vi "GpuMat Create.vi"(8 "error in (no error)":errorcluster) -> (0 "error out":errorcluster, 3 "GpuMat out":refnum<class "GpuMat.lvclass">)   [LabVIEW 2020, in "OpenLvVision_OpenCv.lvlib" / "Cuda.lvlib" / "GpuMat.lvclass"]
doc: "Object by reference!\n\nInitializes an empty `GpuMat`. This acts as a default constructor. It does not allocate any GPU memory; it simply creates the header structure. The matrix will have 0 rows and 0 columns, and its `.empty()` method will return true until data is uploaded or allocated to it."
uses:
  GpuMat.lvclass
  C:/Users/lukas/Documents/OpenLvVision_OpenCv/SourceCode/LabView/OpenLvVision_OpenCv/_LvHelpers/EdvrObject/EdvrObject.lvclass
  _LvHelpers/EdvrObject/TypeDef/Edvr.ctl
  _LvHelpers/EdvrObject/EdvrObject.lvclass/EdvrObject.ctl
  _LvHelpers/EdvrObject/EdvrObject.lvclass
  OpenLvVision_OpenCv.lvlib
  <vilib>/Utility/error.llb/Error Cluster From Error Code.vi
  <vilib>/ErrorRing/Error Ring.xnode
  Dlls/OlvOpenCvWrapper.dll
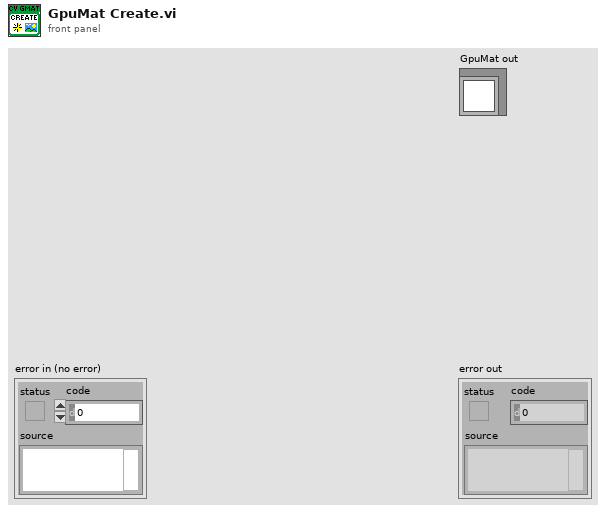
[diagram p1: front panel]
types:
  T1 = typedef "OpenLvVision_OpenCv.lvlib/EdvrObject.lvclass/Edvr.ctl" = refnum<data-value>
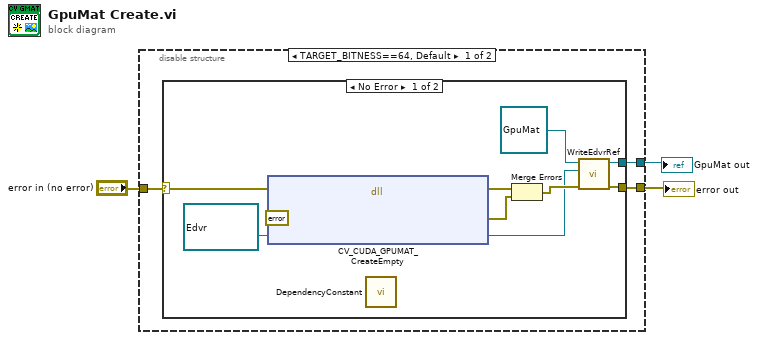
[diagram p0: block diagram]
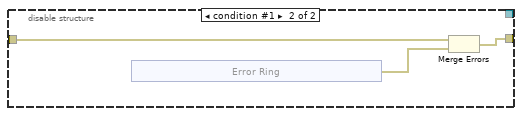
[diagram p3: hidden frame]
diagram:
  n1 = disable-structure shown="TARGET_BITNESS==64, Default" {
    disable-tunnel: "error in (no error)" -> [w6 w19]
    disable-tunnel: [w5 _] -> w2
    disable-tunnel: [w4 w20] -> w3
    frame condition #0 (active) {
      n2 = case shown="No Error" w6 {
        selector: w6 -> [w9 w17]
        tunnel: [w16 w17] -> w4
        tunnel: [w15 _] -> w5
        frame No Error {
          n3 = dll-call lib="C:/Users/lukas/Documents/OpenLvVision_OpenCv/SourceCode/LabView/OpenLvVision_OpenCv/Dlls/OlvOpenCvWrapper.dll" fn="CV_CUDA_GPUMAT_CreateEmpty"(error in=w9, "Error"=errorcluster {"status"=FALSE, "code"=0, "source"=""} ("error out"), "edvrRef"=T1 refnum ("Edvr")) -> (error out=w13:errorcluster, "Error"=w12:errorcluster, "edvrRef"=w8:T1)  [unwired: 3 in, 1 out]
          n4 = call "DependencyConstant.vi"() -> ()  [unwired: 12 in]
          n5 = Merge Errors(w13, w12) -> (w10:errorcluster)
          n6 = call "WriteEdvrRef.vi"("error in (no error)"=w10, "Edvr"=w8, "EdvrObject in"=refnum<class "GpuMat.lvclass"> refnum ("OpenLvVision_OpenCv.lvlib:Cuda:GpuMat")) -> ("error out"=w16:errorcluster, "EdvrObject out"=w15:refnum<class "GpuMat.lvclass">)  [unwired: 7 in]
        }
        frame Error {
        }
      }
    }
    frame condition #1 {
      n7 = xnode "Error Ring"() -> ("error out"=w18:errorcluster)
      n8 = Merge Errors(w19, w18) -> (w20:errorcluster)
    }
  }
  "error out" <- w3
  "GpuMat out" <- w2
